vi "Create Session.vi"(5 "Session in":refnum<class "Session.lvclass">, 8 "error in (no error)":errorcluster, 9 "Request":refnum<queue>, 11 "Connection":refnum<class "Connection.lvclass">) -> (0 "error out":errorcluster, 3 "Session":refnum<class "Session.lvclass">)   [LabVIEW 2013, in "MQTT Base.lvlib" / "Session.lvclass"]
uses:
  Session.lvclass
  <vilib>/LabVIEW Open Source Project/Connection/Connection/Connection.lvclass
  Base Class/Request -- cluster.ctl
  <vilib>/LabVIEW Open Source Project/MQTT Control Packets/Control Packets/ControlPacket/ControlPacket.lvclass
  Base Class/Response -- cluster.ctl
  Session State -- cluster.ctl
  <vilib>/LabVIEW Open Source Project/MQTT Control Packets/Control Packets/SUBSCRIBE/Topic Subscription -- cluster.ctl
  <vilib>/LabVIEW Open Source Project/MQTT Control Packets/Control Packets/ControlPacket/QualityOfService -- enum.ctl
  <vilib>/LabVIEW Open Source Project/MQTT Control Packets/Control Packets/ControlPacket/Pending Transmission -- cluster.ctl
  MQTT_Connection/Connection/Connection.lvclass
  MQTT_Connection/Connection/Connection.lvclass/Connection.ctl
  Session.lvclass/Session.ctl
  DebuggingTerminal/DebuggingTerminal.lvclass
  Base Class/MQTT_Base.lvclass
  <vilib>/LabVIEW Open Source Project/MQTT Control Packets/Control Packets/SUBSCRIBE/SUBSCRIBE.lvclass
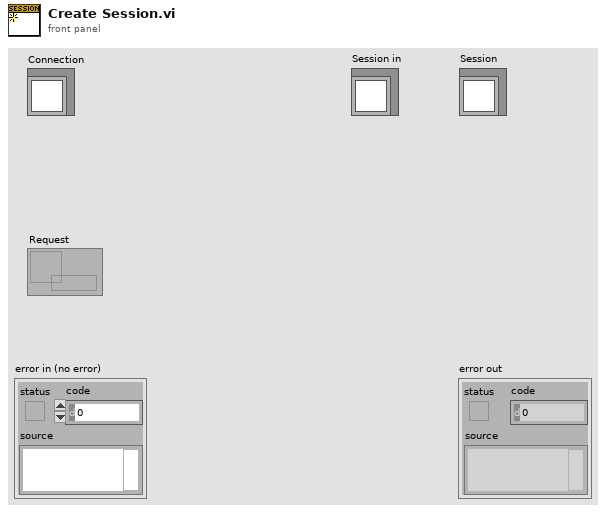
[diagram p1: front panel]
types:
  T1 = typedef "MQTT Base.lvlib/MQTT_Base.lvclass/Response -- cluster.ctl" = cluster{"Packet":refnum<class "ControlPacket.lvclass">, "Protocol Error":errorcluster, "disconnect session":bool, "[ACK]":refnum<notifier>[]}
  T2 = typedef "MQTT Base.lvlib/Session.lvclass/Session State -- cluster.ctl" = cluster{"CleanSession":bool, "Client ID":string, "Subscriptions":T3[], "Pending Transmissions":T5[], "Pending ACK map":variant}
  T3 = typedef "MQTT_Control_Packets.lvlib/SUBSCRIBE.lvclass/Topic Subscription -- cluster.ctl" = cluster{"Topic Filter":string, "QoS":T4}
  T4 = typedef "MQTT_Control_Packets.lvlib/ControlPacket.lvclass/QualityOfService -- enum.ctl" = enum16{"0 (At Most Once)", "1 (At Least Once)", "2 (Exactly Once)"}
  T5 = typedef "MQTT_Control_Packets.lvlib/ControlPacket.lvclass/Pending Transmission -- cluster.ctl" = cluster{"Message":refnum<class "ControlPacket.lvclass">, "QoS":T4, "Tx-Rx":bool}
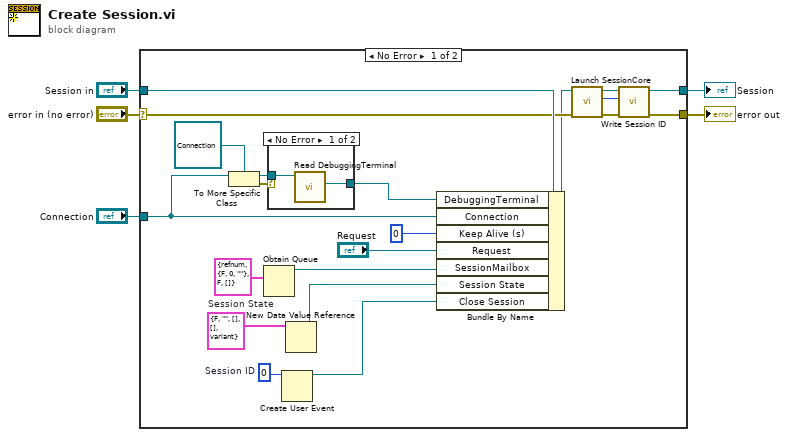
[diagram p0: block diagram]
diagram:
  n1 = case shown="No Error" "error in (no error)" {
    selector: "error in (no error)" -> [w21 w29]
    tunnel: [w15 w29] -> w4
    tunnel: [w20 w28] -> w2
    tunnel: "Session in" -> [w24 w28]
    tunnel: "Connection" -> [w10 _]
    frame No Error {
      w13 = 0  # Session ID
      w19 = T2 {"CleanSession"=FALSE, "Client ID"="", "Subscriptions"=[], "Pending Transmissions"=[], "Pending ACK map"=variant}  # Session State
      n2 = To More Specific Class(target class=refnum<class "Connection.lvclass"> refnum ("MQTT_Connection.lvlib:Connection.lvclass"), reference=w10) -> (specific class reference=w8:refnum<class "Connection.lvclass">, error out=w6:errorcluster)  [unwired: 1 in]
      n3 = Obtain Queue(element data type=T1 {"Packet"=refnum, "Protocol Error"={"status"=FALSE, "code"=0, "source"=""}, "disconnect session"=FALSE, "[ACK]"=[]} ("Response")) -> (queue out=w25:refnum<queue>)  [unwired: 4 in, 2 out]
      n4 = case shown="No Error" w6 {
        tunnel: w8 -> [w27 _]
        tunnel: [w26 _] -> w7
        frame No Error {
          n5 = call "Read DebuggingTerminal.vi"("Connection in"=w27) -> ("DebuggingTerminal"=w26:refnum<class "DebuggingTerminal.lvclass">)  [unwired: 9 in, 1 out]
        }
        frame Error {
        }
      }
      n6 = Create User Event(user event datatype=w13) -> (user event=w12:refnum<user-event>)  [unwired: 1 in, 1 out]
      n7 = New Data Value Reference(data value=w19) -> (data value reference=w18:refnum<data-value>)  [unwired: 1 in, 1 out]
      n8 = Bundle By Name(cluster=w24, "DebuggingTerminal"=w7, "Connection"=w10, "Keep Alive (s)"=0, "Request"="Request", "SessionMailbox"=w25, "Session State"=w18, "Close Session"=w12) -> (w14:refnum<class "Session.lvclass">)
      n9 = call "Launch SessionCore.vi"("error in (no error)"=w21, "Session in"=w14) -> ("error out"=w15:errorcluster, "Session ID"=w17:i32, "Session out"=w16:refnum<class "Session.lvclass">)  [unwired: 7 in]
      n10 = call "Write Session ID.vi"("Session ID"=w17, "Session in"=w16) -> ("Session out"=w20:refnum<class "Session.lvclass">)  [unwired: 8 in, 1 out]
    }
    frame Error {
    }
  }
  "error out" <- w4
  "Session" <- w2
